vi "Main Page.vi"(8 "error in (no error)":errorcluster, 11 "Node Ptr":T1 format="%.0x") -> (0 "error out":errorcluster)   [LabVIEW 2020, in "NI-SWITCH System Explorer.lvlib"]
uses:
  NI-SWITCH System Explorer.lvlib
  <vilib>/NI VeriStand/Custom Device API/Custom Device Item Ref.ctl
  Main Page Controls.ctl
  <vilib>/NI VeriStand/Custom Device API/Custom Device API.lvlib
  Scripting/NI-SWITCH Scripting.lvlib
  Shared/UI Common/UI Common.lvlib
panel:
  out "Normally Connected Information":cluster{"String":string}={"String"="This topology contains endpoints which are normally connected. See the documentation for more information."}
  in  "Custom Device Name":string
  in  "Topology":string(combo)
  in  "Resource":string
  in  "SHDocVw.IWebBrowser":refnum<k7>(container)
  in  "Description":string
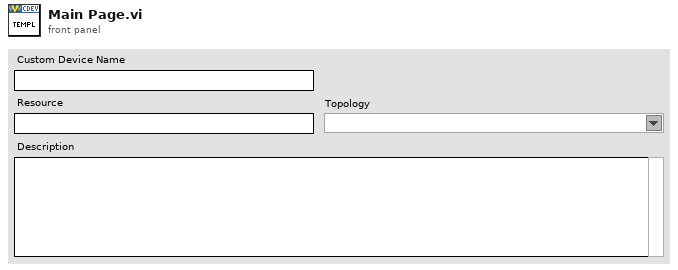
[diagram p1: front panel]
types:
  T1 = typedef "Custom Device API.lvlib/Custom Device Item Ref.ctl" = u64
  T2 = typedef "NI-SWITCH System Explorer.lvlib/Main Page Controls.ctl" = cluster{"Name":refnum<vi>, "Description":refnum<vi>, "Resource":refnum<vi>, "Topology":refnum<vi>, "Normally Connected Information":refnum<vi>}
  T3 = typedef "Custom Device API.lvlib/Custom Device Commands.ctl" = enum16{"Default", "Item renamed", "Shutdown", "Dynamic button pressed"}
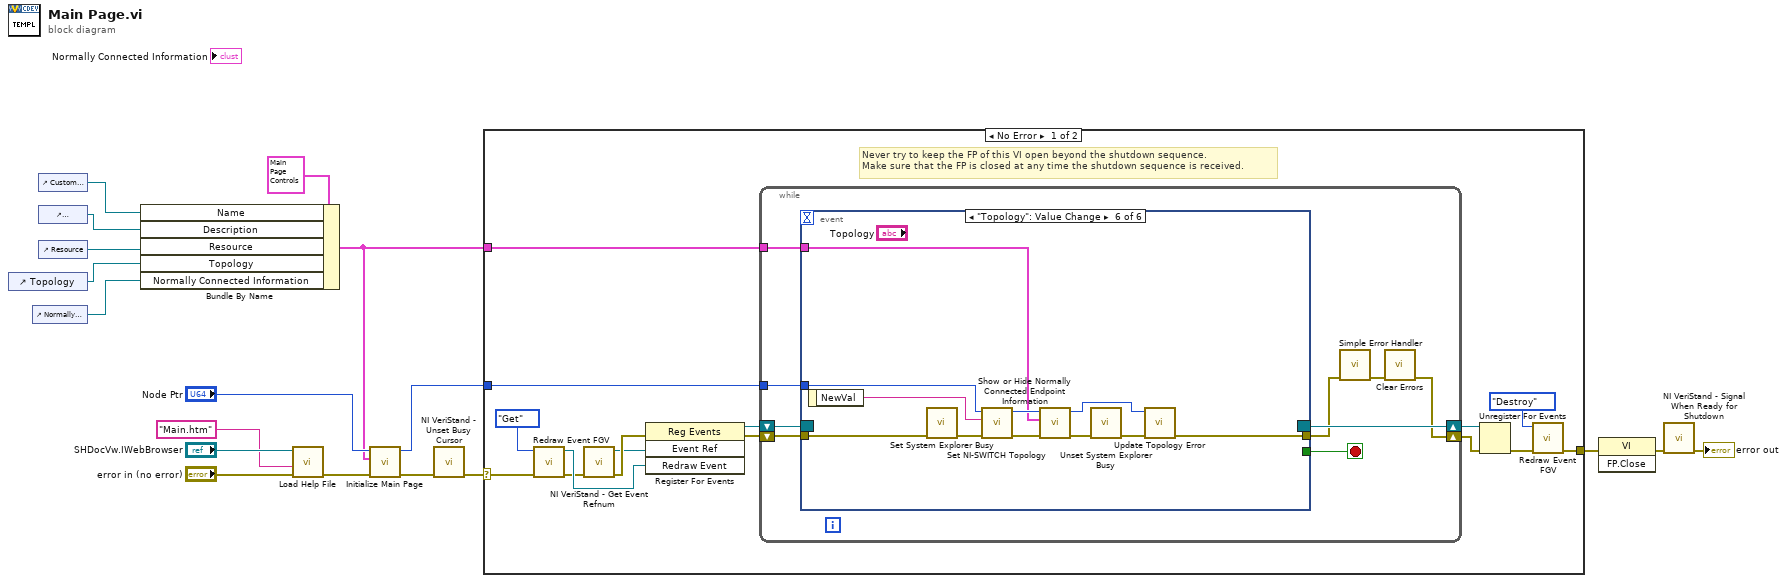
[diagram p0: block diagram]
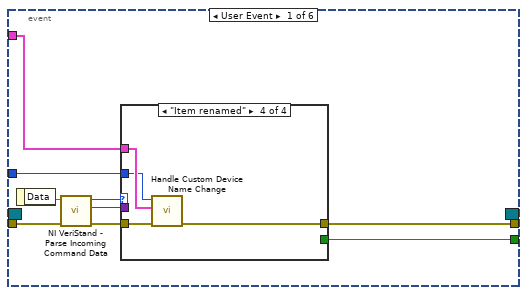
[diagram p2: hidden frame]
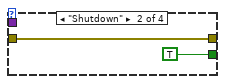
[diagram p4: hidden frame]
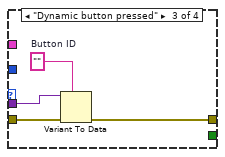
[diagram p5: hidden frame]
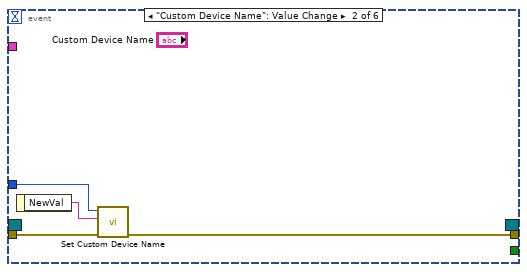
[diagram p6: hidden frame]
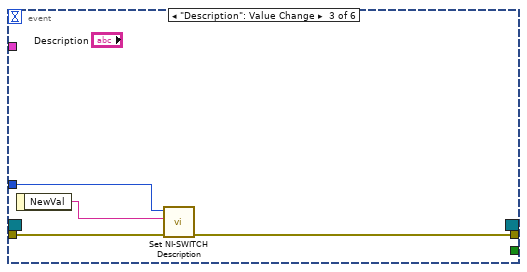
[diagram p7: hidden frame]
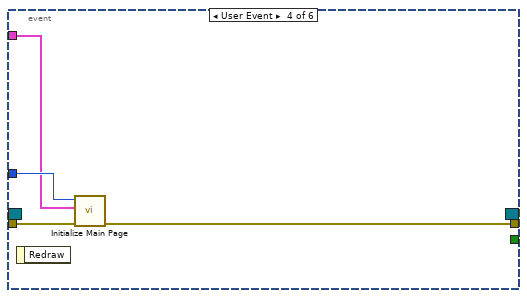
[diagram p8: hidden frame]
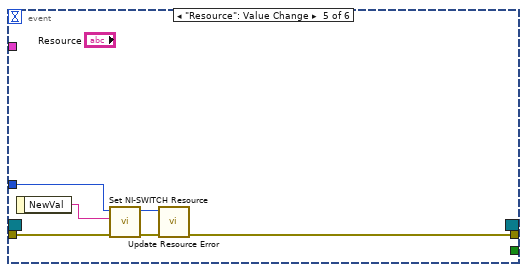
[diagram p9: hidden frame]
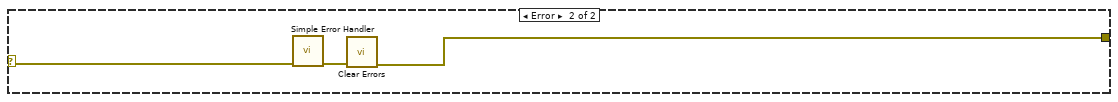
[diagram p10: hidden frame]
diagram:
  n1 = control-ref of="Topology"() -> (w5:refnum<vi>)
  n2 = control-ref of="Normally Connected Information"() -> (w1:refnum<vi>)
  n3 = control-ref of="Custom Device Name"() -> (w2:refnum<vi>)
  n4 = control-ref of="Description"() -> (w8:refnum<vi>)
  n5 = control-ref of="Resource"() -> (w4:refnum<vi>)
  n6 = Bundle By Name(cluster=T2 {"Name"=refnum, "Description"=refnum, "Resource"=refnum, "Topology"=refnum, "Normally Connected Information"=refnum} ("Main Page Controls"), "Name"=w2, "Description"=w8, "Resource"=w4, "Topology"=w5, "Normally Connected Information"=w1) -> (w3:T2)
  n7 = call "Load Help File.vi"("error in (no error)"="error in (no error)", "HTML File to Load"="Main.htm" ("HTML File"), "Browser"="SHDocVw.IWebBrowser") -> ("error out"=w6:errorcluster)  [unwired: 8 in]
  n8 = call "Initialize Main Page.vi"("error in (no error)"=w6, "Main Page Controls"=w3, "Item Ref in"="Node Ptr") -> ("error out"=w14:errorcluster, "Item Ref out"=w11:T1)  [unwired: 7 in]
  n9 = call <vilib>:"NI VeriStand - Unset Busy Cursor.vi"("error in (no error)"=w14) -> ("error out"=w13:errorcluster)  [unwired: 10 out]
  n10 = case shown="No Error" w13 {
    selector: w13 -> [w21 w94]
    tunnel: [w23 w92] -> w18
    tunnel: w11 -> [w27 _]
    tunnel: w3 -> [w25 _]
    frame No Error {
      # "Never try to keep the FP of this VI open beyond the shutdown sequence.\nMake sure that the FP is closed at any time the shutdown sequence is received."
      n11 = call "Redraw Event FGV.vi"("error in (no error)"=w21, "Action (Get)"=enum16{"Get", "Destroy"}."Get") -> ("error out"=w20:errorcluster, "Redraw Event"=w26:refnum<user-event>)  [unwired: 8 in]
      n12 = call <vilib>:"NI VeriStand - Get Event Refnum.vi"("error in (no error)"=w20) -> ("error out"=w33:errorcluster, "Event Ref"=w30:refnum<user-event>)  [unwired: 9 out]
      n13 = register-events(error in=w33, w30, w26) -> (reference out=w28:refnum<event-registration>, error out=w29:errorcluster)  [unwired: 1 in]
      n14 = while {
        tunnel: w27 -> [w38]
        shift-right: [w35] -> w31
        shift-left: w29 -> [w41]
        shift-right: [w42] -> w32
        shift-left: w28 -> [w40]
        tunnel: w25 -> [w34]
        stop <- w39 stop-if-true
        n15 = event shown="[5] \"Topology\": Value Change" {
          selector: w40 -> [_ _ _ _ _ _]
          dyn-events: [_ _ _ _ _ _] -> w42
          timeout: _ -> [_ _ _ _ _ _]
          tunnel: w41 -> [w51 w66 w69 w72 w80 w91]
          tunnel: [w47 _ _ _ _ _] -> w39
          tunnel: [w46 w65 w68 w71 w75 w82] -> w37
          tunnel: w38 -> [w45 w64 w70 w74 w79 w90]
          tunnel: w34 -> [w43 _ _ w73 _ w85]
          event User Event {
            n16 = event-data() -> ("Data"=w50:string)  [unwired: 1 out]
            n17 = call <vilib>:"NI VeriStand - Parse Incoming Command Data.vi"("error in (no error)"=w51, "Incoming data"=w50) -> ("error out"=w49:errorcluster, "Outgoing data"=w44:variant, "Action"=w48:T3)  [unwired: 7 out]
            n18 = case shown="\"Item renamed\"" w48 {
              tunnel: w49 -> [w52 w53 w58 w62]
              tunnel: [_ TRUE _ _] -> w47
              tunnel: [w52 w53 w55 w61] -> w46
              tunnel: w45 -> [_ _ _ w59]
              tunnel: w44 -> [_ _ w57 _]
              tunnel: w43 -> [_ _ _ w60]
              frame "Default", Default {
              }
              frame "Shutdown" {
              }
              frame "Dynamic button pressed" {
                w56 = ""  # Button ID
                n19 = Variant To Data(error in=w58, type=w56, Variant=w57) -> (error out=w55:errorcluster)  [unwired: 1 out]
              }
              frame "Item renamed" {
                n20 = call "Handle Custom Device Name Change.vi"("error in (no error)"=w62, "Main Page Controls"=w60, "Item Ref in"=w59) -> ("error out"=w61:errorcluster)  [unwired: 7 in, 1 out]
              }
            }
          }
          event "Custom Device Name": Value Change {
            n21 = event-data() -> ("NewVal"=w63:string)  [unwired: 1 out]
            n22 = call "Set Custom Device Name.vi"("error in"=w66, "name"=w63, "ni-switch custom device in"=w64) -> ("error out"=w65:errorcluster)  [unwired: 6 in, 1 out]
          }
          event "Description": Value Change {
            n23 = event-data() -> ("NewVal"=w67:string)  [unwired: 1 out]
            n24 = call "Set NI-SWITCH Description.vi"("error in"=w69, "description"=w67, "ni-switch custom device in"=w70) -> ("error out"=w68:errorcluster)  [unwired: 7 in, 1 out]
          }
          event User Event {
            n25 = event-data() -> ()  [unwired: 2 out]
            n26 = call "Initialize Main Page.vi"("error in (no error)"=w72, "Main Page Controls"=w73, "Item Ref in"=w74) -> ("error out"=w71:errorcluster)  [unwired: 7 in, 1 out]
          }
          event "Resource": Value Change {
            n27 = event-data() -> ("NewVal"=w78:string)  [unwired: 1 out]
            n28 = call "Set NI-SWITCH Resource.vi"("error in"=w80, "resource"=w78, "ni-switch custom device in"=w79) -> ("error out"=w77:errorcluster, "ni-switch custom device out"=w76:T1)  [unwired: 7 in]
            n29 = call "Update Resource Error.vi"("error in"=w77, "ni-switch custom device in"=w76) -> ("error out"=w75:errorcluster)  [unwired: 8 in, 1 out]
          }
          event "Topology": Value Change {
            n30 = event-data() -> ("NewVal"=w89:string)  [unwired: 1 out]
            n31 = call "Set System Explorer Busy.vi"("error in (no error)"=w91) -> ("error out"=w84:errorcluster)  [unwired: 10 in]
            n32 = call "Set NI-SWITCH Topology.vi"("error in"=w84, "topology"=w89, "ni-switch custom device in"=w90) -> ("error out"=w88:errorcluster, "ni-switch custom device out"=w86:T1)  [unwired: 7 in]
            n33 = call "Show or Hide Normally Connected Endpoint Information.vi"("error in (no error)"=w88, "Main Page Controls"=w85, "ni-switch custom device in"=w86) -> ("error out"=w87:errorcluster, "ni-switch custom device out"=w81:T1)  [unwired: 7 in]
            n34 = call "Unset System Explorer Busy.vi"("error in (no error)"=w87) -> ("error out"=w83:errorcluster)  [unwired: 10 in]
            n35 = call "Update Topology Error.vi"("error in"=w83, "ni-switch custom device in"=w81) -> ("error out"=w82:errorcluster)  [unwired: 8 in, 1 out]
          }
        }
        n36 = call <vilib>:"Simple Error Handler.vi"("error in (no error)"=w37) -> ("error out"=w36:errorcluster)  [unwired: 1 in, 7 out]
        n37 = call <vilib>:"Clear Errors.vi"("error in (no error)"=w36) -> ("error out"=w35:errorcluster)  [unwired: 1 in, 5 out]
      }
      n38 = Unregister For Events(event registration refnum=w32, error in=w31) -> (error out=w24:errorcluster)
      n39 = call "Redraw Event FGV.vi"("error in (no error)"=w24, "Action (Get)"=enum16{"Get", "Destroy"}."Destroy") -> ("error out"=w23:errorcluster)  [unwired: 8 in, 1 out]
    }
    frame Error {
      n40 = call <vilib>:"Simple Error Handler.vi"("error in (no error)"=w94) -> ("error out"=w93:errorcluster)  [unwired: 1 in, 7 out]
      n41 = call <vilib>:"Clear Errors.vi"("error in (no error)"=w93) -> ("error out"=w92:errorcluster)  [unwired: 1 in, 5 out]
    }
  }
  n42 = invoke class="VI" method="FP.Close"(error in=w18) -> (error out=w17:errorcluster)  [unwired: 2 in, 2 out]
  n43 = call <vilib>:"NI VeriStand - Signal When Ready for Shutdown.vi"("error in (no error)"=w17) -> ("error out"=→"error out":errorcluster)  [unwired: 10 out]
